vi "Remove Subscription.vi"(8 "error in (no error)":errorcluster, 9 "Topic Filter":string, 10 "SessionMailbox":refnum<queue>, 11 "MQTT Server":refnum<class "Server.lvclass">) -> (0 "error out":errorcluster, 1 "Done":bool, 3 "MQTT Server":refnum<class "Server.lvclass">)   [LabVIEW 2013, in "MQTT Server.lvlib" / "Server.lvclass"]
uses:
  Server.lvclass
  <vilib>/LabVIEW Open Source Project/MQTT Connection/MQTT_Base/Base Class/Response -- cluster.ctl
  <vilib>/LabVIEW Open Source Project/MQTT Control Packets/Control Packets/ControlPacket/ControlPacket.lvclass
  Server.lvclass/Server.ctl
  Subscription/_Subscription.lvclass/_Subscription.ctl
  TopicFilter/_TopicFilter.lvclass/_TopicFilter.ctl
  Subscription/_Subscription.lvclass
  StoredSessions/StoredSessions.lvclass
  <vilib>/LabVIEW Open Source Project/MQTT Connection/MQTT_Base/Base Class/MQTT_Base.lvclass
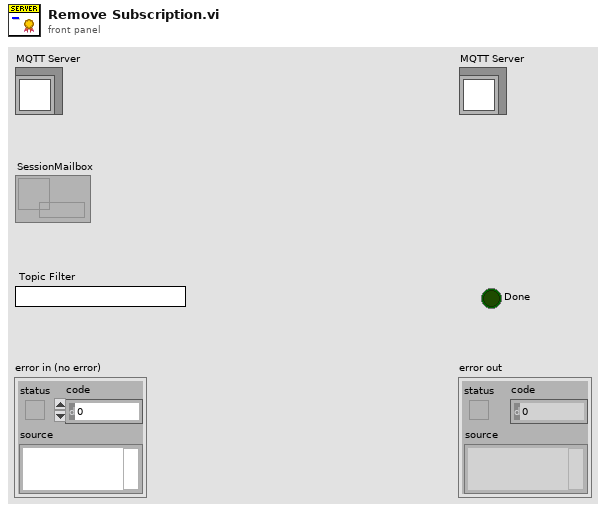
[diagram p1: front panel]
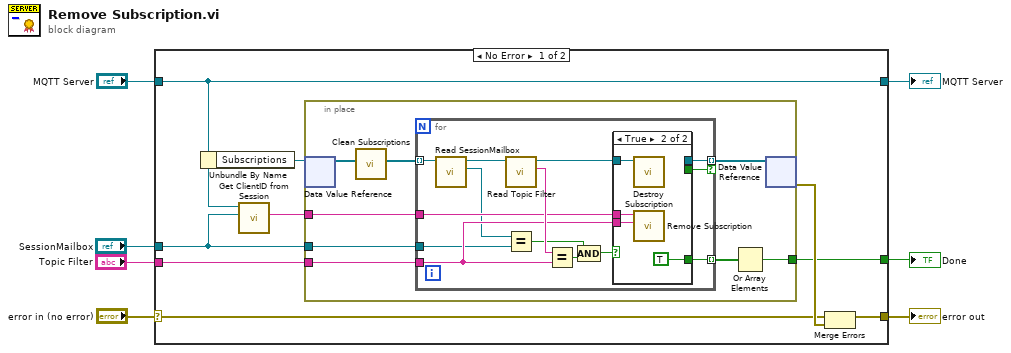
[diagram p0: block diagram]
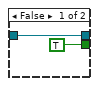
[diagram p2: hidden frame]
diagram:
  n1 = case shown="No Error" "error in (no error)" {
    selector: "error in (no error)" -> [w14 w46]
    tunnel: [w13 w46] -> w6
    tunnel: [w10 w45] -> w4
    tunnel: "MQTT Server" -> [w10 w45]
    tunnel: "SessionMailbox" -> [w9 _]
    tunnel: [w12 _] -> w2
    tunnel: "Topic Filter" -> [w11 _]
    frame No Error {
      n2 = Unbundle By Name(w10) -> ("Subscriptions"=w16:refnum<data-value>)
      n3 = call "Get ClientID from Session.vi"("SessionMailbox"=w9, "MQTT Server"=w10) -> ("Client ID"=w8:string)  [unwired: 6 in, 3 out]
      n4 = in-place {
        in-place-border: w9 -> [w24]
        in-place-border: [w22] -> w12
        in-place-border: w11 -> [w18]
        in-place-border: w8 -> [w19]
        n5 = in-place-dvr #1(w16) -> (w21:refnum<class "_Subscription.lvclass">[])  [unwired: 1 out]
        n6 = call "Clean Subscriptions.vi"("Subscriptions in"=w21) -> ("Subscriptions"=w20:refnum<class "_Subscription.lvclass">[])  [unwired: 10 in]
        n7 = for {
          tunnel: w19 -> [w35]
          tunnel: w18 -> [w34]
          tunnel: w24 -> [w31]
          tunnel: w20 -> [w29] mode=indexing
          tunnel: [w27] -> w23 mode=indexing if=w26
          tunnel: [w25] -> w17 mode=indexing
          n8 = call "Read SessionMailbox.vi"("Subscription in"=w29) -> ("SessionMailbox"=w32:refnum<queue>, "Subscription out"=w33:refnum<class "_Subscription.lvclass">)  [unwired: 8 in, 1 out]
          n9 = call "Read Topic Filter.vi"("Subscription in"=w33) -> ("Topic Filter"=w38:string, "Subscription out"=w36:refnum<class "_Subscription.lvclass">)  [unwired: 7 in, 2 out]
          n10 = Equal?(x=w32, y=w31) -> (x = y?=w30:bool)
          n11 = Equal?(x=w38, y=w34) -> (x = y?=w37:bool)
          n12 = Compound Arithmetic op=AND(w30, w37) -> (w28:bool)
          n13 = case shown="True" w28 {
            tunnel: w36 -> [w40 w44]
            tunnel: w35 -> [_ w43]
            tunnel: w34 -> [_ w42]
            tunnel: [w40 _] -> w27
            tunnel: [TRUE _] -> w26
            tunnel: [_ TRUE] -> w25
            frame False {
            }
            frame True {
              n14 = call "Destroy Subscription.vi"("Subscription in"=w44) -> ()  [unwired: 9 in, 2 out]
              n15 = call "Remove Subscription.vi"("Topic Filter"=w42, "Client ID"=w43) -> ()  [unwired: 9 in, 1 out]
            }
          }
        }
        n16 = Or Array Elements(Boolean array=w17) -> (logical OR=w22:bool)
        n17 = in-place-dvr #1(w23) -> (w15:errorcluster)  [unwired: 1 out]
      }
      n18 = Merge Errors(w14, w15) -> (w13:errorcluster)
    }
    frame Error {
    }
  }
  "error out" <- w6
  "MQTT Server" <- w4
  "Done" <- w2
